vi "Delete Wire.vi"(0 "terminal reference":refnum<vi>, 11 "error in":errorcluster) -> (15 "error out":errorcluster)   [LabVIEW 2021, in "Converter.lvlib"]
uses:
  Converter.lvlib
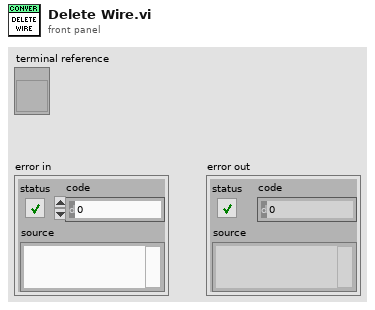
[diagram p1: front panel]
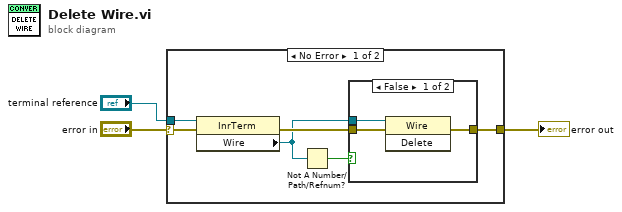
[diagram p0: block diagram]
diagram:
  n1 = case shown="No Error" "error in" {
    selector: "error in" -> [w9 w14]
    tunnel: [w5 w14] -> w3
    tunnel: "terminal reference" -> [w6 _]
    frame No Error {
      n2 = property class="InrTerm"(reference=w6, error in=w9) -> (error out=w8:errorcluster, "Wire"=w7:refnum<vi>)  [unwired: 1 out]
      n3 = Not A Number/Path/Refnum?(number/path/refnum=w7) -> (NaN/Path/Refnum?=w4:bool)
      n4 = case shown="False" w4 {
        tunnel: w7 -> [w12 _]
        tunnel: w8 -> [w11 w13]
        tunnel: [w10 w13] -> w5
        frame False {
          n5 = invoke class="Wire" method="Delete"(reference=w12, error in=w11) -> (error out=w10:errorcluster)  [unwired: 1 in, 2 out]
        }
        frame True {
        }
      }
    }
    frame Error {
    }
  }
  "error out" <- w3
